vi "LaunchCOUI.vi"() -> ()   [LabVIEW 2014]
uses:
  CoordinatorUI_lib/State Pattern UI/CoordinatorUI.lvclass
  Global_var/Global_var.vi
  <vilib>/ActorFramework/Actor/Actor.lvclass
panel:
  in  "Ini_maxvel":dbl=0.4 format="%#_13g"
  in  "模拟":bool
  in  "address":string="192.168.31.68"
  out "error out":errorcluster caption="错误输出"
  # "笔记本：192.168.31.133; 192.168.1.117"
  # "机器人：192.168.31.68; 192.168.1.134"
  # "笔记本：192.168.31.127"
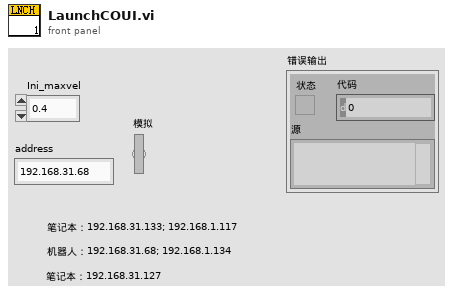
[diagram p1: front panel]
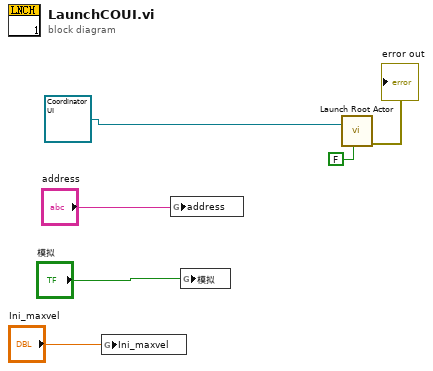
[diagram p0: block diagram]
diagram:
  n1 = global write "Global_var.vi" "Ini_maxvel"("Ini_maxvel") -> ()
  n2 = global write "Global_var.vi" "address"("address") -> ()
  n3 = global write "Global_var.vi" "模拟"("模拟") -> ()
  n4 = call <vilib>:"Launch Root Actor.vi"("Open Actor Core front panel? (F)"=FALSE, "Actor"=refnum<class "CoordinatorUI.lvclass"> refnum ("CoordinatorUI.lvlib:CoordinatorUI.lvclass")) -> ("error out"=→"error out":errorcluster)  [unwired: 8 in, 1 out]
